vi "Launch uService.vi"(4 "Highlander?":bool, 6 "uService ID":string, 8 "error in (no error)":errorcluster, 9 "GUI?":bool, 10 "uService Class Name":string, 11 "Guardian in":refnum<class "Guardian.lvclass">) -> (0 "error out":errorcluster, 3 "Guardian out":refnum<class "Guardian.lvclass">)   [LabVIEW 2020, in "TALOS.lvlib" / "Guardian.lvlib" / "Guardian.lvclass"]
doc: "This VI get called everytime a uService has to be launched. The optional uService ID input is needed if a different name is wanted for a specific uService, otherwise the class name is used (useful when launching more than an instance of a uService, for example)."
uses:
  Guardian.lvclass
  C:/LabVIEW Code/TALOS/talos/Ancestor/Ancestor/Ancestor.lvclass
  C:/LabVIEW Code/TALOS/builds/Actor Framework PPL/Actor Framework.lvlibp/1abvi3w/vi.lib/ActorFramework/Actor/Actor.lvclass
  Classes/uService List/uService Properties.ctl
  builds/Actor Framework PPL/Actor Framework.lvlibp/1abvi3w/vi.lib/ActorFramework/Message Enqueuer/Message Enqueuer.lvclass
  Ancestor/Ancestor/Ancestor.lvclass/Ancestor.ctl
  Classes/uService List/uService List.lvclass/uService List.ctl
  Guardian Messages/Broadcast to Guardians Msg/Broadcast to Guardians Msg.lvclass/Broadcast to Guardians Msg.ctl
  Guardian.lvclass/Guardian.ctl
  Ancestor/Ancestor/Read Distr uS Map ref.vi
  Ancestor/Ancestor/Write Distr uS Map ref.vi
  Ancestor/Ancestor/Read ID.vi
  Support VIs/Generate Error.vi
  FGV/Error Memory/Get Error Description.vi
  Support VIs/Get PC name.vi
  Support VIs/Get Class Name.vi
  <vilib>/Utility/error.llb/Clear Errors.vi
  FGV/Error Memory/Error Memory Core.vi
  <vilib>/AdvancedString/Delimited String to 1D String Array.vi
  Support VIs/Circus Root Path.vi
  FGV/Error Memory/Error Crt Lvl checker.vi
  FGV/Error Memory/Error Memory Core.vi/40c8088d-b597-4017-91af-faa98e00292e.vi
  FGV/Error Memory/Error Memory Core.vi/d4a3ab98-063c-4e44-b43d-fbdcfe6c2be2.vi
  Father of all uServices/Father of all uServices/Father of all uServices.lvclass
  builds/Actor Framework PPL/Actor Framework.lvlibp/1abvi3w/vi.lib/ActorFramework/Message Enqueuer/Enqueue.vi
  Support VIs/Global Memory.vi
  <vilib>/Utility/LVClass/Get LV Class Name.vi
  Support VIs/Is in Packed Library.vi
  Support VIs/TALOS Root path.vi
  Support VIs/Read CSV worksheet.vi
  Support VIs/Global Constants.vi
  <vilib>/Utility/error.llb/General Error Handler.vi
  Support VIs/Error Log.vi
  Classes/uService List/uService List.lvclass
  Classes/Distributed uService Map/Distributed uService Map.lvclass
  Guardian Messages/Broadcast to Guardians Msg/Broadcast to Guardians Msg.lvclass
  Ancestor/Ancestor/Ancestor.lvclass
  <vilib>/Comparison/Equal/Equal Functor/Equal Functor.lvclass
  builds/Actor Framework PPL/Actor Framework.lvlibp/1abvi3w/vi.lib/ActorFramework/Actor/Actor.lvclass
  TALOS.lvlib
  C:/LabVIEW Code/TALOS/talos/Guardian/Guardian/Guardian.lvclass
  C:/LabVIEW Code/TALOS/talos/Father of all uServices/Father of all uServices/Father of all uServices.lvclass
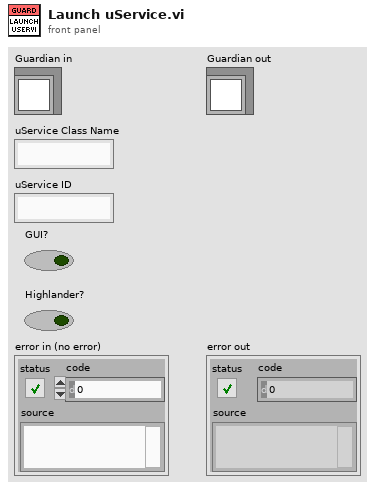
[diagram p1: front panel]
types:
  T1 = typedef "TALOS.lvlib/Classes.lvlib/uService List.lvclass/uService Properties.ctl" = cluster{"uService Queue":refnum<class "Message Enqueuer.lvclass">, "Last Pat":timestamp, "Online":bool, "Vi Ref":refnum<vi>, "Class name":string, "GUI":bool, "FP Items Refs Map":map{string, refnum<vi>}, "Remote GUI":bool, "Remote Window":refnum<vi>}
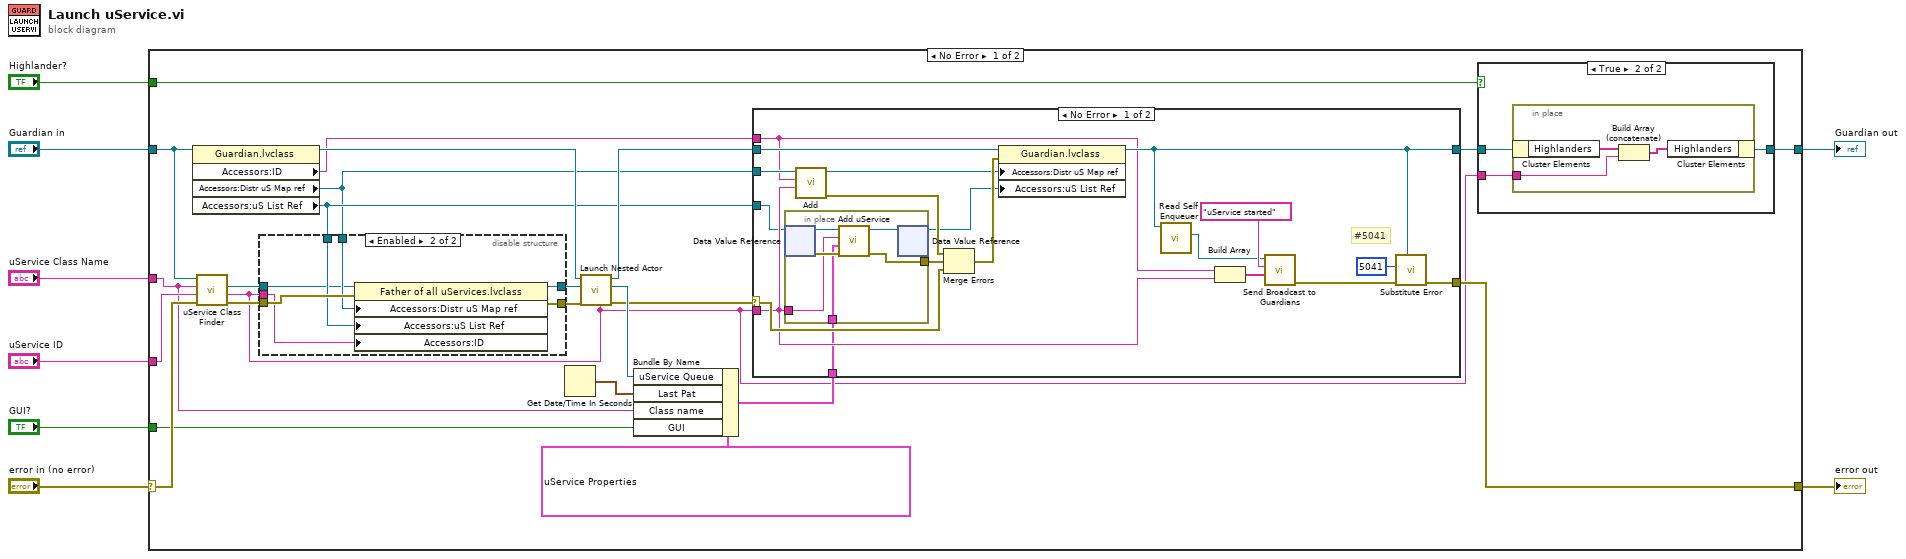
[diagram p0: block diagram]
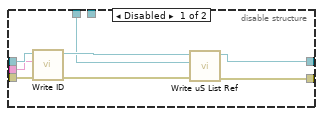
[diagram p2: hidden frame]
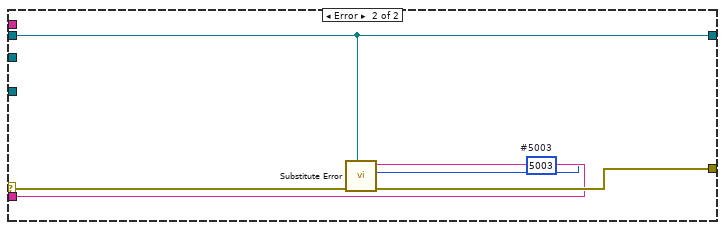
[diagram p3: hidden frame]
diagram:
  n1 = case shown="No Error" "error in (no error)" {
    selector: "error in (no error)" -> [w31 w85]
    tunnel: "Guardian in" -> [w18 w86]
    tunnel: "uService Class Name" -> [w17 _]
    tunnel: [w16 w85] -> w5
    tunnel: [w13 w86] -> w4
    tunnel: "GUI?" -> [w27 _]
    tunnel: "uService ID" -> [w20 _]
    tunnel: "Highlander?" -> [w14 _]
    frame No Error {
      n2 = property class="Guardian.lvclass"(reference=w18) -> (reference out=w25:refnum<class "Guardian.lvclass">, "Accessors:ID"=w11:string, "Accessors:Distr uS Map ref"=w9:refnum<data-value>, "Accessors:uS List Ref"=w12:refnum<data-value>)  [unwired: 1 in, 1 out]
      n3 = call "uService Class Finder.vi"("error in (no error)"=w31, "uService ID in"=w20, "uService Class name"=w17, "Guardian in"=w18) -> ("error out"=w32:errorcluster, "uService ID out"=w10:string, "uService out"=w19:refnum<class "Father of all uServices.lvclass">)  [unwired: 4 in, 1 out]
      n4 = disable-structure shown="Enabled" {
        disable-tunnel: w32 -> [w40 w47]
        disable-tunnel: [w37 w41] -> w24
        disable-tunnel: [w36 w46] -> w23
        disable-tunnel: w19 -> [w35 w42]
        disable-tunnel: w10 -> [w34 w45]
        disable-tunnel: w12 -> [w33 w43]
        disable-tunnel: w9 -> [_ w44]
        frame Disabled {
          n5 = call "Write ID.vi"("error in (no error)"=w40, "ID"=w34, "Ancestor in"=w35) -> ("error out"=w38:errorcluster, "Ancestor out"=w39:refnum<class "Father of all uServices.lvclass">)  [unwired: 7 in]
          n6 = call "Write uS List Ref.vi"("error in (no error)"=w38, "uS List Ref"=w33, "Ancestor in"=w39) -> ("error out"=w36:errorcluster, "Ancestor out"=w37:refnum<class "Father of all uServices.lvclass">)  [unwired: 7 in]
        }
        frame Enabled {
          n7 = property class="Father of all uServices.lvclass"(reference=w42, error in=w47, "Accessors:Distr uS Map ref"=w44, "Accessors:uS List Ref"=w43, "Accessors:ID"=w45) -> (reference out=w41:refnum<class "Father of all uServices.lvclass">, error out=w46:errorcluster)
        }
      }
      n8 = Get Date/Time In Seconds() -> (seconds since 1Jan1904=w30:timestamp)
      n9 = call "Launch Nested Actor.vi"("Debug Alias"=w10, "error in (no error)"=w23, "Nested Actor"=w24, "Caller Actor in"=w25) -> ("error out"=w21:errorcluster, "Nested Actor's Enqueuer"=w29:refnum<class "Message Enqueuer.lvclass">, "Caller Actor out"=w26:refnum<class "Guardian.lvclass">)  [unwired: 5 in]
      n10 = Bundle By Name(cluster=T1 {"uService Queue"=refnum, "Last Pat"=timestamp(0 s since 1904-01-01), "Online"=FALSE, "Vi Ref"=refnum, "Class name"="", "GUI"=FALSE, "FP Items Refs Map"={}, "Remote GUI"=FALSE, "Remote Window"=refnum} ("uService Properties"), "uService Queue"=w29, "Last Pat"=w30, "Class name"=w17, "GUI"=w27) -> (w22:T1)
      n11 = case shown="No Error" w21 {
        selector: w21 -> [w66 w77]
        tunnel: w26 -> [w62 w75]
        tunnel: w12 -> [w61 _]
        tunnel: w22 -> [w60 _]
        tunnel: w10 -> [w65 w74]
        tunnel: [w52 w75] -> w15
        tunnel: [w54 w76] -> w16
        tunnel: w11 -> [w48 _]
        tunnel: w9 -> [w50 _]
        frame No Error {
          # "#5041"
          n12 = in-place {
            in-place-border: w60 -> [w70]
            in-place-border: w65 -> [w69]
            in-place-border: [w68] -> w59
            n13 = in-place-dvr #1(w61) -> (w71:refnum<class "uService List.lvclass">, w72:errorcluster)
            n14 = call "Add uService.vi"("error in (no error)"=w72, "uService Properties"=w70, "ID"=w69, "uService List in"=w71) -> ("error out"=w68:errorcluster, "uService List out"=w67:refnum<class "uService List.lvclass">)  [unwired: 6 in]
            n15 = in-place-dvr #1(w67) -> (w51:refnum<data-value>)  [unwired: 1 out]
          }
          n16 = call "Add.vi"("uService"=w65, "Guardian"=w48, "Distr uS Map ref in"=w50) -> ("error out"=w64:errorcluster, "Distr uS Map ref out"=w49:refnum<data-value>)  [unwired: 6 in, 1 out]
          n17 = Merge Errors(w64, w59, w66) -> (w63:errorcluster)
          n18 = property class="Guardian.lvclass"(reference=w62, error in=w63, "Accessors:Distr uS Map ref"=w49, "Accessors:uS List Ref"=w51) -> (reference out=w52:refnum<class "Guardian.lvclass">)  [unwired: 1 out]
          n19 = call "Read Self Enqueuer.vi"("Actor"=w52) -> ("Self Enqueuer"=w56:refnum<class "Message Enqueuer.lvclass">)  [unwired: 10 in]
          n20 = Build Array(w48, w65) -> (w58:string[])
          n21 = call "Send Broadcast to Guardians.vi"("Data"=w58, "Message"="uService started", "Message Enqueuer"=w56) -> ("error out"=w55:errorcluster)  [unwired: 7 in, 1 out]
          n22 = call "Substitute Error.vi"("LabVIEW Object"=w52, "error in (no error)"=w55, "Error Code"=5041) -> ("error out"=w54:errorcluster)  [unwired: 8 in]
        }
        frame Error {
          w73 = 5003  # #5003
          n23 = call "Substitute Error.vi"("LabVIEW Object"=w75, "error in (no error)"=w77, "Error Code"=w73, "Optional String"=w74) -> ("error out"=w76:errorcluster)  [unwired: 7 in]
        }
      }
      n24 = case shown="True" w14 {
        tunnel: w15 -> [w78 w81]
        tunnel: w10 -> [_ w80]
        tunnel: [w78 w79] -> w13
        frame False {
        }
        frame True {
          n25 = in-place {
            in-place-border: w80 -> [w83]
            n26 = in-place-cluster #2(w81) -> ("Highlanders"=w84:string[])
            n27 = Build Array (concatenate)(w84, w83) -> (w82:string[])
            n28 = in-place-cluster #2("Highlanders"=w82) -> (w79:refnum<class "Guardian.lvclass">)
          }
        }
      }
    }
    frame Error {
    }
  }
  "error out" <- w5
  "Guardian out" <- w4
